vi "Simulated_Robot_Diff_Drive.vi"() -> ()   [LabVIEW 2019]
doc: "This WebSockets API example VI acts as a server for an incoming websockets connection. Receives/sends string data to the connected client."
uses:
  <vilib>/Rock Robotics/WPI/Simulation/Protocol/Devices/PWM/PWM proto.ctl
  <vilib>/Rock Robotics/WPI/Simulation/Protocol/Devices/PWM/PWM data proto.ctl
  <vilib>/Rock Robotics/WPI/Simulation/Protocol/Devices/RoboRIO/RoboRIO proto.ctl
  <vilib>/Rock Robotics/WPI/Simulation/Protocol/Devices/RoboRIO/RoboRIO data proto.ctl
  <vilib>/Rock Robotics/WPI/Simulation/Protocol/Devices/DriverStation/DS proto.ctl
  <vilib>/Rock Robotics/WPI/Simulation/Protocol/Devices/DriverStation/DS data proto.ctl
  <vilib>/Rock Robotics/WPI/Simulation/Protocol/Devices/Gyro/Gyro proto.ctl
  <vilib>/Rock Robotics/WPI/Simulation/Protocol/Devices/Gyro/Gyro Data proto.ctl
  <vilib>/Rock Robotics/WPI/Simulation/Protocol/Devices/Encoder/Encoder proto.ctl
  <vilib>/Rock Robotics/WPI/Simulation/Protocol/Devices/Encoder/Encoder data protoo.ctl
  <vilib>/Rock Robotics/WPI/ThirdParty/JAS_Junk/TrajLib/TypeDef/DIFF_DRIVE_TRAIN_SIM.ctl
  <vilib>/Rock Robotics/WPI/ThirdParty/JAS_Junk/TrajLib/TypeDef/LINEAR_SYSTEM.ctl
  <vilib>/Analysis/Matrix/Datatypes/RealMatrix.ctl
  <vilib>/Rock Robotics/WPI/ThirdParty/JAS_Junk/TrajLib/TypeDef/DCMOTOR.CTL
  <vilib>/vision/Image Controls.llb/IMAQ Image.ctl
  Simulated_Field/Simulated_Field_ROBOT_PICTURE.ctl
  DiffDriveSim/DiffDriveSim_PhysRobotInfoType.ctl
  DiffDriveSim/DiffDriveSim_KitBotDriveInfoType.ctl
  <vilib>/Rock Robotics/WPI/ThirdParty/JAS_Junk/TrajLib/Enum/DIFF_DRIVE_ToughBoxMini_MotorChoice_ENUM.ctl
  <vilib>/Rock Robotics/WPI/ThirdParty/JAS_Junk/TrajLib/Enum/DIFF_DRIVE_KitBot_WheelSize_ENUM.ctl
  <vilib>/Rock Robotics/WPI/ThirdParty/JAS_Junk/TrajLib/Enum/DIFF_DRIVE_ToughBoxMini_GearChoice_ENUM.ctl
  DiffDriveSim/DiffDriveSim_CustomDriveIntoType.ctl
  <vilib>/Rock Robotics/WPI/ThirdParty/JAS_Junk/TrajLib/Enum/DCMOTOR_TYPES_ENUM.ctl
  DiffDriveSim/DiffDriveSim_EncoderDIOType.ctl
  <vilib>/Rock Robotics/SystemInterfaces/DIO/FPGA_DIOChannel.ctl
  <vilib>/Rock Robotics/SystemInterfaces/DIO/FPGA_DIOPWMChannel.ctl
  <vilib>/Utility/miscctls.llb/LVBoundsTypeDef.ctl
  <vilib>/Rock Robotics/WPI/Simulation/Protocol/Devices/RoboRIO/RoboRIO Update Ops.ctl
  <vilib>/Rock Robotics/WPI/Simulation/Protocol/Devices/DriverStation/DS Update Ops.ctl
  <vilib>/Rock Robotics/WPI/ThirdParty/JAS_Junk/TrajLib/Rotation2d_CreateAngle.vi
  <vilib>/Rock Robotics/WPI/ThirdParty/JAS_Junk/TrajLib/Translation2d_Create.vi
  <vilib>/Rock Robotics/WPI/ThirdParty/JAS_Junk/TrajLib/MathUtil_Clamp.vi
  <vilib>/Rock Robotics/WPI/ThirdParty/JAS_Junk/TrajLib/BatterySim_CalculateLoadedBatteryVoltage.vi
  Simulated_Field/Simulated_Field_FIELD_ODOM_CLAMP.vi
  DiffDriveSim/DiffDriveSim_ClampFieldPosition.vi
  <vilib>/Rock Robotics/WPI/ThirdParty/JAS_Junk/TrajLib/Conv_Meters_Feet.vi
  DiffDriveSim/DiffDriveSim_FindEncoder.vi
  DiffDriveSim/DiffDriveSim_GetAllEncoderInx.vi
  <vilib>/Rock Robotics/SystemInterfaces/FPGA_NIFPGAInterfaceFPGAResourceConstant.vi
  <vilib>/MediaMongrels Ltd/WebSockets/WebSockets/WebSocket Server/WebSocket Server.lvclass
  C:/Program Files/National Instruments/LabVIEW 2019/vi.lib/MediaMongrels Ltd/WebSockets/WebSockets/WebSocket/WebSocket.lvclass
  Simulated_Robot_Globals.vi
  <vilib>/picture/pixmap.llb/Flatten Pixmap.vi
  <vilib>/picture/pictutil.llb/Create Mask.vi
  <vilib>/picture/picture.llb/Draw Flattened Pixmap.vi
  <vilib>/Rock Robotics/WPI/ThirdParty/JAS_Junk/TrajLib/DiffDriveTrainSim_SetInputs.vi
  <vilib>/Rock Robotics/WPI/ThirdParty/JAS_Junk/TrajLib/DiffDriveTrainSim_Update.vi
  <vilib>/Rock Robotics/WPI/ThirdParty/JAS_Junk/TrajLib/DiffDriveTrainSim_GetPose.vi
  <vilib>/Rock Robotics/WPI/ThirdParty/JAS_Junk/TrajLib/DiffDriveTrainSim_GetCurrentDrawAmps.vi
  <vilib>/Rock Robotics/WPI/ThirdParty/JAS_Junk/TrajLib/DiffDriveTrainSim_GetLeftVelocityMetersPerSecond.vi
  <vilib>/Rock Robotics/WPI/ThirdParty/JAS_Junk/TrajLib/DiffDriveTrainSim_GetRightPositionMeters.vi
  <vilib>/Rock Robotics/WPI/ThirdParty/JAS_Junk/TrajLib/DiffDriveTrainSim_GetLeftPositionMeters.vi
  <vilib>/Rock Robotics/WPI/ThirdParty/JAS_Junk/TrajLib/DiffDriveTrainSim_GetHeading.vi
  <vilib>/Rock Robotics/WPI/ThirdParty/JAS_Junk/TrajLib/DiffDriveTrainSim_GetRightVelocityMetersPerSecond.vi
  Simulated_Field/Simulated_Field.lvlib
  <vilib>/Rock Robotics/WPI/ThirdParty/JAS_Junk/TrajLib/Trajectory_Library.lvlib
  <vilib>/Rock Robotics/WPI/Simulation/Protocol/Devices/PWM/PWM Update Ops.ctl
  <vilib>/Rock Robotics/WPI/Simulation/Protocol/Devices/Gyro/Gyro Update Ops.ctl
  <vilib>/Rock Robotics/WPI/Simulation/Protocol/Devices/Encoder/Encoder Update Ops.ctl
  <vilib>/Analysis/Matrix/NI_Matrix.lvlib
panel:
  in  "Tab Control":T1(tab)
  out "Simulation\n  Running":bool
  in  "Start Simulation":bool
  in  "Field Selector":string(combo)
  in  "Robot Y Position\nInches":dbl=84.0
  in  "Robot X Position\nInches":dbl=120.0
  in  "Robot Orientation\nDegrees":dbl
  in  "Custom Drive Info":T2={"Motor Type"=enum."CIM", "Num Motors Per Side"=1, "Wheel Diameter Inch"=7.0, "Gear Ratio"=1.0} {"Gear Ratio" format="%#_13g"; "Wheel Diameter Inch" format="%#_13g"}
  in  "Robot Physical Info":T4={"Mass_LB"=80.0, "Actual TrackWidth Inch"=26.0, "Skid Factor"=1.75} {"Actual TrackWidth Inch" format="%#_13g"}
  in  "KitBot Drive Info":T5={"ToughBoxMiniMotor"=enum."One CIM Per Side", "Wheelsize"=enum."6 Inch", "ToughBoxMiniGear"=enum."Ratio_8_45"}
  in  "Use Custom Drive":bool
  in  "Encoder Counts/Rev":dbl=360.0
  in  "Left Drive Encoder":T9={"Enc A DI Channel"=enum."DIO 4", "Enc B DI Channel"=enum."DIO 5"}
  in  "Right Drive Encoder":T9={"Enc A DI Channel"=enum."DIO 6", "Enc B DI Channel"=enum."DIO 7"}
  in  "Left Drive Motor":T11
  in  "Right Drive Motor":T11=enum."PWM 1"
  out "Simulation\n  Running":bool
  out "Right Dist Ft":dbl format="%15.1f"
  out "Left Dist Ft":dbl format="%15.1f"
  out "Heading Deg":dbl format="%11.1f"
  out "Right Wheel\nFt / Sec":dbl format="%11.1f"
  out "Left Wheel\nFt / Sec":dbl format="%11.1f"
  out "RSL ON":picture
  out "ROBOT":T12
  out "RSL OFF":picture
  out "Field Picture":picture
  out "Y Pos Inch":dbl format="%11.1f"
  out "X Pos Inch":dbl format="%11.1f"
  out "Gyro":T13={"type"="Gyro", "device"="", "name"="", "data"={"<init"=0, ">connected"=FALSE, "<offsetX"=0.0, "<offsetY"=0.0, "<offsetZ"=0.0, ">angle_x"=0.0, ">angle_y"=0.0, ">angle_z"=0.0, ">rate_x"=0.0, ">rate_y"=0.0, ">rate_z"=0.0, "<gain"=0.0}}
  out "Enc Left":T15={"type"="Encoder", "device"="", "name"="", "data"={"<init"=FALSE, ">count"=0.0, ">period"=0.0, "<samples_to_avg"=0, "<offset"=0.0, "<channel_a"=0, "<channel_b"=0}}
  out "Enc Right":T15={"type"="Encoder", "device"="", "name"="", "data"={"<init"=FALSE, ">count"=0.0, ">period"=0.0, "<samples_to_avg"=0, "<offset"=0.0, "<channel_a"=0, "<channel_b"=0}}
  out "PWM 0":T17
  out "PWM 1":T17
  out "roboRIO":T19={"type"="roboRIO", "device"="", "name"="", "data"={">fpga_button"=FALSE, ">vin_voltage"=0.0, ">vin_current"=0.0, ">6v_voltage"=0.0, ">6v_current"=0.0, ">6v_active"=FALSE, ">6v_faults"=0.0, ">5v_voltage"=0.0, ">5v_current"=0.0, ">5v_active"=FALSE, ">5v_faults"=0.0, ">3v3_voltage"=0.0, ">3v3_current"=0.0, ">3v3_active"=FALSE, ">3v3_faults"=0.0}}
  out "Driverstation":T21={"type"="Driverstation", "device"="", "name"="", "data"={">enabled"=FALSE, ">autonomous"=FALSE, ">test"=FALSE, ">estop"=FALSE, ">fms"=FALSE, ">ds"=FALSE, "<match_time"=0.0, ">station"="", ">game_data"=""}}
  out "Request URI":string
  out "HTTP Headers":variant
  out "No Robot Comm":bool
  out "Battery Voltage VDC":dbl format="%18.2f"
  out "Gyro Reading   Deg":dbl format="%19.3f"
  out "Edges/Feet":dbl
  out "out DiffDriveTrainSim":T23 {"m_Motor"."Jr_KgM2" format="%13.5p"; "m_Motor"."L_H" format="%13.5p"; "m_Motor"."Kt_NMPerAmp" format="%13.5p"; "m_Motor"."KvINV_RadPerSecPerVolt" format="%13.5p"; "m_Motor"."R_Ohms" format="%13.5p"; "m_Motor"."FreeSpeed_RadPerSec" format="%13.5p"; "m_Motor"."FreeCurrent_Amps" format="%13.5p"; "m_Motor"."StallCurrent_Amps" format="%13.5p"; "m_Motor"."StallTorque_NM" format="%13.5p"; "m_Motor"."nominalVoltage_Volts" format="%13.5p"}
  out "Speed Left  Ft/Sec":dbl format="%13.2f"
  out "Speed Right  Ft/Sec":dbl format="%13.2f"
  out "Amps":dbl
  out "PWM 0 Rate":dbl format="%19.3f"
  out "PWM 1 Rate":dbl format="%19.3f"
  out "FIeld Image":T27
  out "Y Pos Pixel":dbl format="%11.1f"
  out "X Pos Pixel":dbl format="%11.1f"
  in  "Restart":bool
  out "Ctrl Loop Offset MS":dbl
  out "Robot Enabled":bool
  # "Robot Position"
  # "Robot Speed / Distance"
  # "<States, 1>"
  # "<Outputs, 1>"
  # "<Inputs, 1>"
  # "<Outputs, 1>"
  # "<States,States>"
  # "<States,Inputs>"
  # "<Outputs,States>"
  # "<Outputs,Inputs>"
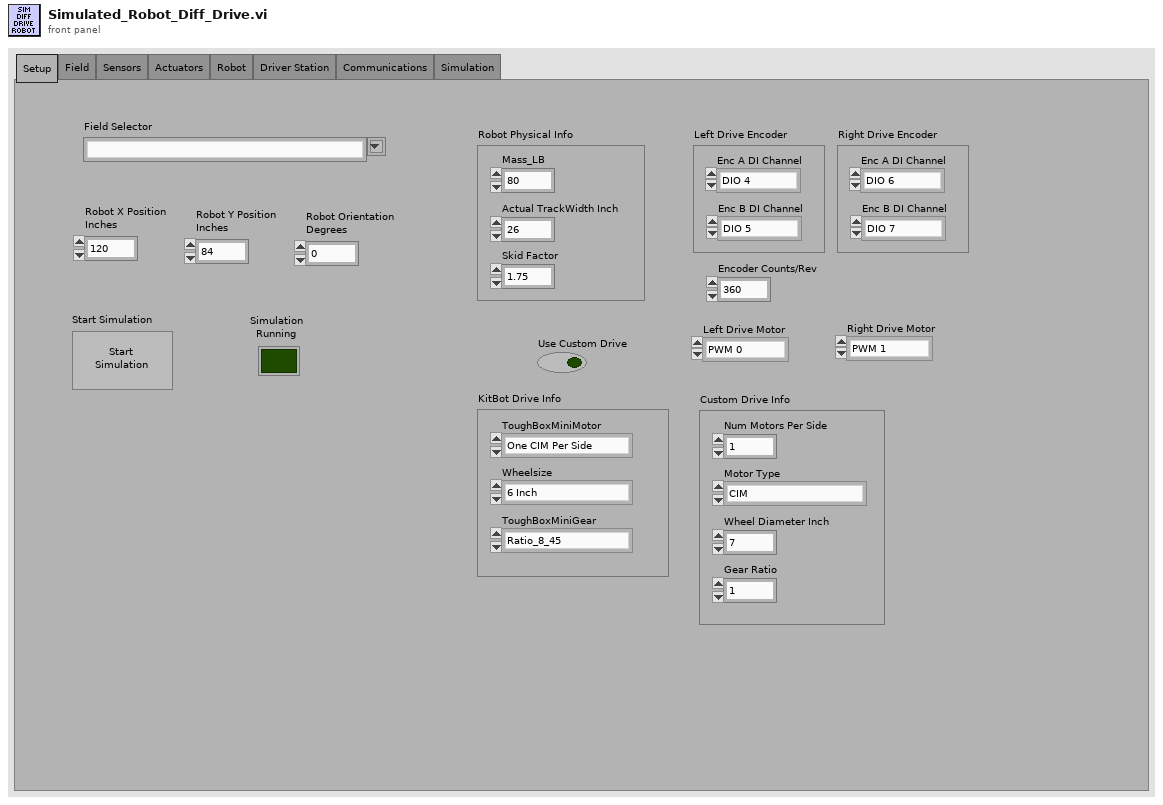
[diagram p1: front panel]
types:
  T1 = enum32{"Setup", "Field", "Sensors", "Actuators", "Robot", "Driver Station", "Communications", "Simulation"}
  T2 = typedef "DiffDriveSim_CustomDriveIntoType.ctl" = cluster{"Motor Type":T3, "Num Motors Per Side":i32, "Wheel Diameter Inch":dbl, "Gear Ratio":dbl}
  T3 = typedef "Trajectory_Library.lvlib/DCMOTOR_TYPES_ENUM.ctl" = enum16{"CIM", "AndyMark 9015", "Andy Mark RS 775 125", "Bag", "BaneBots RS 550", "BaneBots RS 775", "Falcon 500", "Mini CIM", "NEO", "NEO 550", "Romi BuiltIn", "Vex 775 Pro"}
  T4 = typedef "DiffDriveSim_PhysRobotInfoType.ctl" = cluster{"Mass_LB":dbl, "Actual TrackWidth Inch":dbl, "Skid Factor":dbl}
  T5 = typedef "DiffDriveSim_KitBotDriveInfoType.ctl" = cluster{"ToughBoxMiniMotor":T6, "Wheelsize":T7, "ToughBoxMiniGear":T8}
  T6 = typedef "Trajectory_Library.lvlib/DIFF_DRIVE_ToughBoxMini_MotorChoice_ENUM.ctl" = enum16{"One CIM Per Side", "Two CIM Per Side", "One MiniCIM Per Side", "Two Mini CIM Per Side", "Two Falcon Per Side", "Two NEO Per Side"}
  T7 = typedef "Trajectory_Library.lvlib/DIFF_DRIVE_KitBot_WheelSize_ENUM.ctl" = enum16{"4 Inch", "6 Inch", "8 Inch", "10 Inch"}
  T8 = typedef "Trajectory_Library.lvlib/DIFF_DRIVE_ToughBoxMini_GearChoice_ENUM.ctl" = enum16{"Ratio_12_75", "Ratio_10_71", "Ratio_8_45", "Ratio_7_31", "Ratio_5_95"}
  T9 = typedef "DiffDriveSim_EncoderDIOType.ctl" = cluster{"Enc A DI Channel":T10, "Enc B DI Channel":T10}
  T10 = typedef "FPGA_DIOChannel.ctl" = enum8{"DIO 0", "DIO 1", "DIO 2", "DIO 3", "DIO 4", "DIO 5", "DIO 6", "DIO 7", "DIO 8", "DIO 9", "DIO MXP 0", "DIO MXP 1", "DIO MXP 2", "DIO MXP 3", "DIO MXP 4", "DIO MXP 5", "DIO MXP 6", "DIO MXP 7", "DIO MXP 8", "DIO MXP 9", "DIO MXP 10", "DIO MXP 11", "DIO MXP 12", "DIO MXP 13", "DIO MXP 14", "DIO MXP 15", "SPI Port CS1", "SPI Port CS2", "SPI Port CS3", "SPI Port MISO", "SPI Port MOSI", "Invalid"}
  T11 = typedef "FPGA_DIOPWMChannel.ctl" = enum8{"PWM 0", "PWM 1", "PWM 2", "PWM 3", "PWM 4", "PWM 5", "PWM 6", "PWM 7", "PWM 8", "PWM 9", "PWM MXP 0", "PWM MXP 1", "PWM MXP 2", "PWM MXP 3", "PWM MXP 4", "PWM MXP 5", "PWM MXP 6", "PWM MXP 7", "PWM MXP 8", "PWM MXP 9", "Invalid"}
  T12 = typedef "Simulated_Field.lvlib/Simulated_Field_ROBOT_PICTURE.ctl" = picture
  T13 = typedef "Gyro proto.ctl" = cluster{"type":string, "device":string, "name":string, "data":T14}
  T14 = typedef "Gyro Data proto.ctl" = cluster{"<init":i32, ">connected":bool, "<offsetX":dbl, "<offsetY":dbl, "<offsetZ":dbl, ">angle_x":dbl, ">angle_y":dbl, ">angle_z":dbl, ">rate_x":dbl, ">rate_y":dbl, ">rate_z":dbl, "<gain":dbl}
  T15 = typedef "Encoder proto.ctl" = cluster{"type":string, "device":string, "name":string, "data":T16}
  T16 = typedef "Encoder data protoo.ctl" = cluster{"<init":bool, ">count":dbl, ">period":dbl, "<samples_to_avg":i32, "<offset":dbl, "<channel_a":i32, "<channel_b":i32}
  T17 = typedef "PWM proto.ctl" = cluster{"type":string, "device":string, "name":string, "data":T18}
  T18 = typedef "PWM data proto.ctl" = cluster{"<init":bool, "<speed":dbl, "<position":dbl, "<raw":dbl, "<period_scale":dbl, "<zero_latch":bool, "<servo range":dbl}
  T19 = typedef "RoboRIO proto.ctl" = cluster{"type":string, "device":string, "name":string, "data":T20}
  T20 = typedef "RoboRIO data proto.ctl" = cluster{">fpga_button":bool, ">vin_voltage":dbl, ">vin_current":dbl, ">6v_voltage":dbl, ">6v_current":dbl, ">6v_active":bool, ">6v_faults":dbl, ">5v_voltage":dbl, ">5v_current":dbl, ">5v_active":bool, ">5v_faults":dbl, ">3v3_voltage":dbl, ">3v3_current":dbl, ">3v3_active":bool, ">3v3_faults":dbl}
  T21 = typedef "DS proto.ctl" = cluster{"type":string, "device":string, "name":string, "data":T22}
  T22 = typedef "DS data proto.ctl" = cluster{">enabled":bool, ">autonomous":bool, ">test":bool, ">estop":bool, ">fms":bool, ">ds":bool, "<match_time":dbl, ">station":string, ">game_data":string}
  T23 = typedef "Trajectory_Library.lvlib/DIFF_DRIVE_TRAIN_SIM.ctl" = cluster{"m_Plant":T24, "m_X":T25, "m_Y":T25, "m_U":T25, "MeasureStdDev":T25, "m_Motor":T26, "m_OriginalGearing":dbl, "m_CurrentGearing":dbl, "m_WheelRadius_M":dbl, "m_RB":dbl}
  T24 = typedef "Trajectory_Library.lvlib/LINEAR_SYSTEM.ctl" = cluster{"m_A":T25, "m_B":T25, "m_C":T25, "m_D":T25, "States":i32, "Inputs":i32, "Outputs":i32}
  T25 = typedef "NI_Matrix.lvlib/RealMatrix.ctl" = dbl[][]
  T26 = typedef "Trajectory_Library.lvlib/DCMOTOR.CTL" = cluster{"nominalVoltage_Volts":dbl, "StallTorque_NM":dbl, "StallCurrent_Amps":dbl, "FreeCurrent_Amps":dbl, "FreeSpeed_RadPerSec":dbl, "R_Ohms":dbl, "KvINV_RadPerSecPerVolt":dbl, "Kt_NMPerAmp":dbl, "L_H":dbl, "Jr_KgM2":dbl}
  T27 = typedef "IMAQ Image.ctl" = refnum<image>
  T28 = typedef "LVBoundsTypeDef.ctl" = cluster{"Width":u32, "Height":u32}
  T29 = typedef "Image Type" = u32
  T30 = typedef "Simulated_Field.lvlib/Simulated_Field_Field_Info.ctl" = cluster{"FIeld_File_Name":string, "Top_Left_X":i32, "Top_Left_Y":i32, "Bottom_Right_X":i32, "Bottom_Right_Y":i32, "Field_Size_X":dbl, "Field_Size_Y":dbl, "FIeld_Size_Units":string}
  T31 = typedef "Trajectory_Library.lvlib/POSE2D.ctl" = cluster{"TRANSLATION":T32, "ROTATION":T33}
  T32 = typedef "Trajectory_Library.lvlib/TRANSLATION2D.ctl" = cluster{"X":dbl, "Y":dbl}
  T33 = typedef "Trajectory_Library.lvlib/ROTATION2D.ctl" = cluster{"VALUE":dbl, "COS":dbl, "SIN":dbl}
  T34 = typedef "DS Update Ops.ctl" = enum16{"set enabled", "set autonomous", "set test", "set estop", "set fms", "set ds", "set control word", "set match_time", "set station", "set game data", "JSON update", "set name", "get", "transmit initial", "reset"}
  T35 = typedef "RoboRIO Update Ops.ctl" = enum16{"get", "JSON update", "set name", "transmit initial", "set fpga_button", "set vin_voltage", "set vin_current", "set 6v_voltage", "set 6v_current", "set 6v_active", "set 6v_faults", "set 5v_voltage", "set 5v_current", "set 5v_active", "set 5v_faults", "set 3v3_voltage", "set 3v3_current", "set 3v3_active", "set 3v3_faults", "reset"}
  T36 = typedef "Simulated_Field.lvlib/Simulated_FIeld_Rotated_Picture_TypeDef.ctl" = cluster{"ONE-8-bit pixmap":u8[][], "Two-Array":cdb[][], "Three-Numeric":i32, "Four-Numeric":i32, "Five-Numeric":cdb, "Six-colors":u32[], "Seven-new element/subarray":u32, "Eight-Cluster":cluster{"[0]":i32, "[1]":i32}}
  T37 = typedef "DiffDriveSim_EncoderValues.ctl" = cluster{"Speed Ft/Sec":dbl, "Distance Ft":dbl}
  T38 = typedef "Encoder Update Ops.ctl" = enum16{"set init", "set count", "set period", "set reset", "set samples_to_avg", "get", "delete", "JSON update", "set name", "transmit initial", "reset", "set channel_a", "set channel_b", "set values"}
  T39 = typedef "Gyro Update Ops.ctl" = enum16{"get", "delete", "JSON update", "set  name", "transmit initial", "reset", "set init", "set offsetX", "set offsetY", "set offsetZ", "set gain", "set angle X", "set angle Y", "set angle Z", "set rate X", "set rate Y", "set rate Z"}
  T40 = typedef "PWM Update Ops.ctl" = enum16{"set init", "set speed", "set position", "set raw", "set  period_scale", "set zero_latch", "set angular range", "get", "delete", "JSON update", "set name", "transmit initial", "reset"}
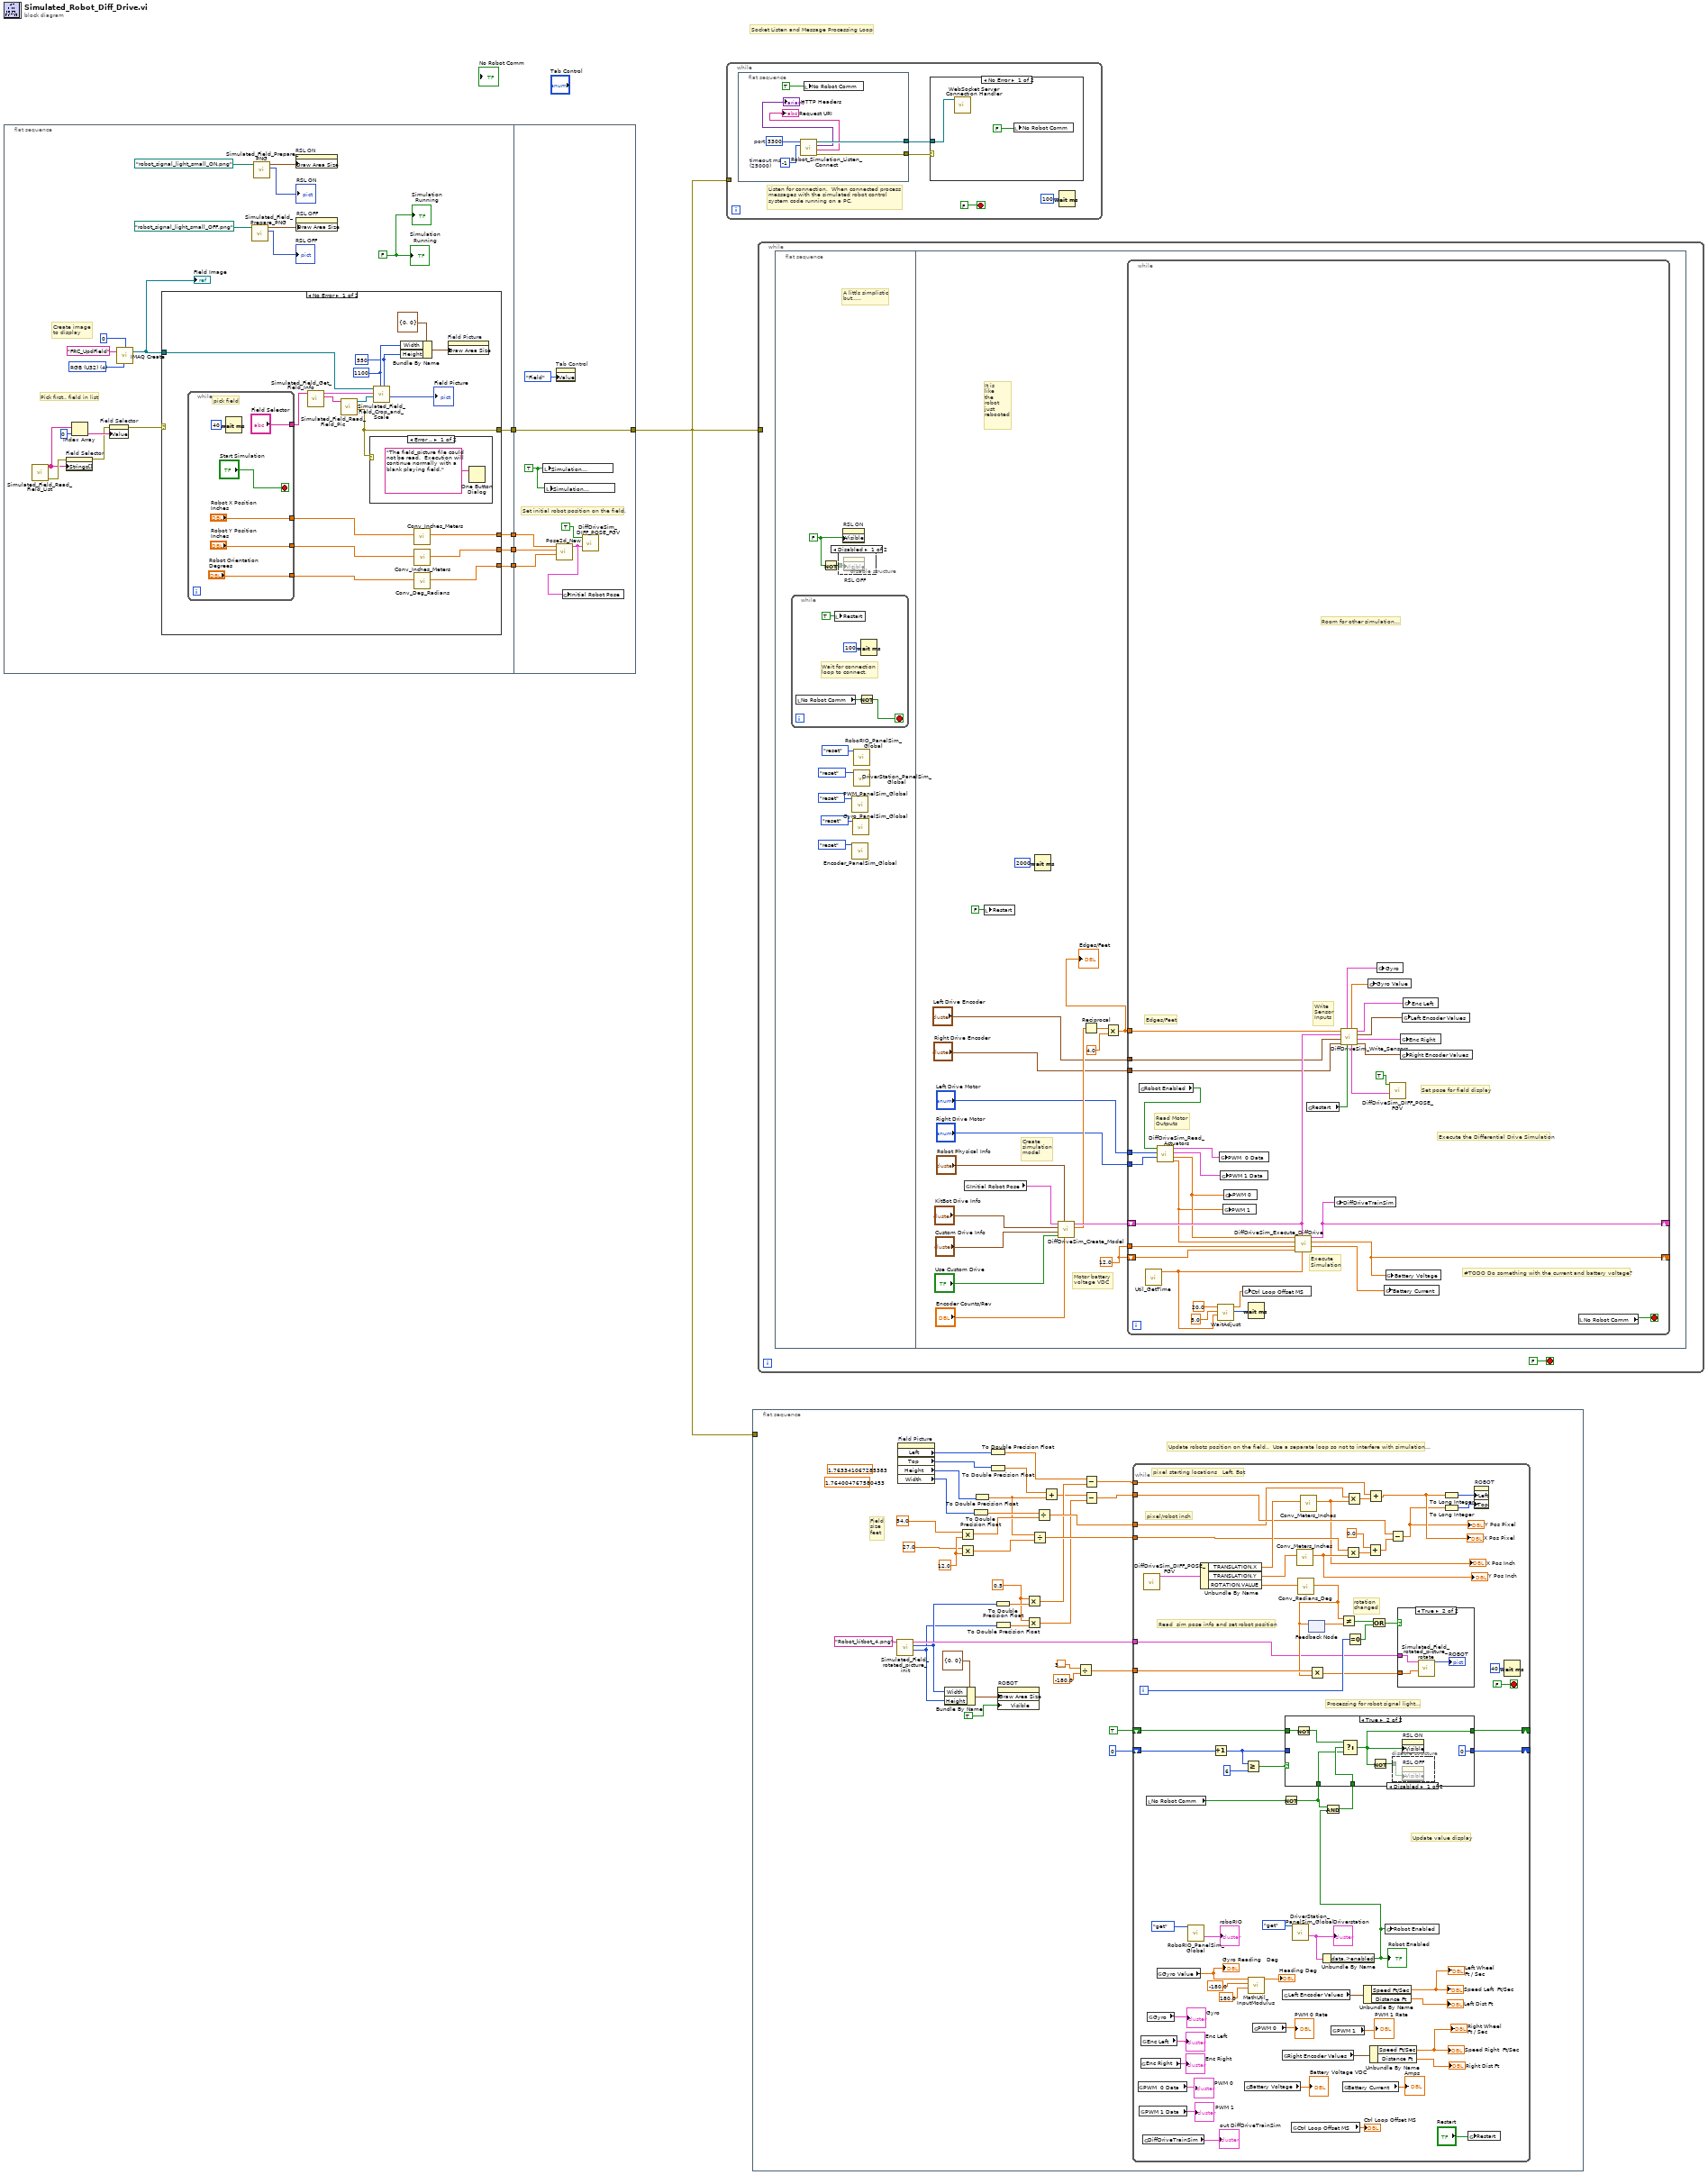
[diagram p0: block diagram]
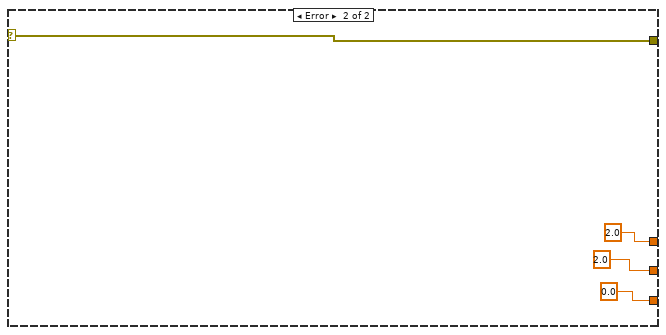
[diagram p6: hidden frame]
diagram:
  # "Socket Listen and Message Processing Loop"
  n1 = flat-sequence {
    tunnel: [w19] -> w5
    tunnel: [w9] -> w3
    tunnel: [w8] -> w2
    tunnel: [w7] -> w1
    tunnel: [w62] -> w4
    tunnel: w5 -> [w62]
    tunnel: w3 -> [w59]
    tunnel: w2 -> [w58]
    tunnel: w1 -> [w57]
    frame #0 {
      w6 = FALSE ("Simulation\n  Running")
      w24 = T29 4 items=["Grayscale (U8)", "Grayscale (I16)", "Grayscale (SGL)", "Complex (CSG)", "RGB (U32)", "HSL (U32)", "RGB (U64)", "Grayscale (U16)"] ("Image Type")
      # "Pick first.. field in list"
      # "Create image \nto display"
      n2 = call "Simulated_Field_Read_Field_List.vi"() -> ("error out"=w15:errorcluster, "section names"=w14:string[])  [unwired: 10 in]
      n3 = property on="Field Selector" class="CmbBox"(error in=w15, "Strings[]"=w14) -> (error out=w11:errorcluster)  [unwired: 1 in, 1 out]
      n4 = Index Array(array=w14, index=0) -> (element=w12:string)
      n5 = property on="Field Selector" class="CmbBox"(error in=w11, "Value"=w12) -> (error out=w10:errorcluster)  [unwired: 1 in, 1 out]
      n6 = call "IMAQ Create"("Border Size"=0, "Image Name"="FRC_UpdField", "Image Type"=w24) -> ("New Image"=w23:T27)  [unwired: 2 in, 1 out]
      "FIeld Image" <- w23
      n7 = case shown="No Error" w10 {
        selector: w10 -> [_ w54]
        tunnel: w23 -> [w34 _]
        tunnel: [w40 w54] -> w19
        tunnel: [w29 2.0 ("Meters")] -> w9
        tunnel: [w28 2.0 ("Meters")] -> w8
        tunnel: [w27 0.0 ("Radians")] -> w7
        frame No Error {
          w35 = 550 ("Disp Y Size Pixel")
          w36 = 1100 ("Disp X Size Pixel")
          n8 = while {
            tunnel: ["Field Selector"] -> w33
            tunnel: ["Robot X Position\nInches"] -> w32
            tunnel: ["Robot Y Position\nInches"] -> w31
            tunnel: ["Robot Orientation\nDegrees"] -> w30
            stop <- "Start Simulation" stop-if-true
            # "pick field"
            n9 = Wait (ms)(milliseconds to wait=u32 40) -> ()  [unwired: 1 out]
          }
          n10 = call "Simulated_Field_Get_Field_Info.vi"("Field Selector"=w33) -> ("File"=w43:string, "input cluster"=w42:T30)  [unwired: 9 in]
          n11 = call "Simulated_Field_Read_Field_Pic.vi"("file name"=w43) -> ("Image Error"=w40:errorcluster, "Image Data"=w41:T27)  [unwired: 7 in, 2 out]
          n12 = case shown="Error .." w40 {
            frame Error {
              n13 = One Button Dialog(message="The field_picture file could not be read.  Execution will continue normally with a blank playing field.") -> ()  [unwired: 1 in, 1 out]
            }
            frame No Error {
            }
          }
          n14 = call "Simulated_Field_Field_Crop_and_Scale.vi"("Disp Y Size Pixel"=w35, "Disp X Size Pixel"=w36, "Field Image"=w41, "field Info"=w42, "Display Image"=w34) -> ("Cropped Field Picture Out"=→"Field Picture":picture)  [unwired: 4 in, 2 out]
          n15 = Bundle By Name(cluster=T28 {"Width"=0, "Height"=0} ("Draw Area Size"), "Width"=w36, "Height"=w35) -> (w37:T28)
          n16 = call <vilib>:"Conv_Inches_Meters.vi"("INCH"=w32) -> ("Meters"=w29:dbl)  [unwired: 10 in]
          n17 = call <vilib>:"Conv_Inches_Meters.vi"("INCH"=w31) -> ("Meters"=w28:dbl)  [unwired: 10 in]
          n18 = call <vilib>:"Conv_Deg_Radians.vi"("Degress"=w30) -> ("Radians"=w27:dbl)  [unwired: 10 in]
          n19 = property on="Field Picture" class="Pict"("Draw Area Size"=w37) -> ()  [unwired: 2 in, 2 out]
        }
        frame Error {
        }
      }
      n20 = call "Simulated_Field_Prepare_PNG.vi"("path to PNG file"=path "robot_signal_light_small_OFF.png") -> ("new picture"=→"RSL OFF":picture, "Draw Area Size"=w18:T28)  [unwired: 9 in]
      n21 = call "Simulated_Field_Prepare_PNG.vi"("path to PNG file"=path "robot_signal_light_small_ON.png") -> ("new picture"=→"RSL ON":picture, "Draw Area Size"=w21:T28)  [unwired: 9 in]
      n22 = property on="RSL ON" class="Pict"("Draw Area Size"=w21) -> ()  [unwired: 2 in, 2 out]
      n23 = property on="RSL OFF" class="Pict"("Draw Area Size"=w18) -> ()  [unwired: 2 in, 2 out]
      "Simulation\n  Running" <- w6
      "Simulation\n  Running" <- w6
    }
    frame #1 {
      w55 = TRUE ("Simulation\n  Running")
      # "Set initial robot position on the field."
      n24 = local write "Simulation\n  Running"(w55) -> ()
      n25 = local write "Simulation\n  Running"(w55) -> ()
      n26 = property on="Tab Control" class="TabCtl (strict)"("Value"=T1."Field" ("Tab Control")) -> ()  [unwired: 2 in, 2 out]
      n27 = call <vilib>:"Pose2d_New.vi"("Heading"=w57, "Y"=w58, "X"=w59) -> ("out POSe"=w56:T31)  [unwired: 8 in]
      n28 = global write "Simulated_Robot_Globals.vi" "Initial Robot Pose"(w56) -> ()
      n29 = call "DiffDriveSim_DIFF_POSE_FGV.vi"("in Sim Pose"=w56, "WRITE"=TRUE) -> ()  [unwired: 9 in, 1 out]
    }
  }
  n30 = while {
    tunnel: w4 -> [_]
    stop <- FALSE stop-if-true
    # "Listen for connection.  When connected process\nmessages with the simulated robot control\nsystem code running on a PC."
    n31 = flat-sequence {
      tunnel: [w71] -> w65
      tunnel: [w69] -> w64
      frame #0 {
        w72 = -1  # timeout ms  (25000)
        w73 = u16 3300  # port
        n32 = call <vilib>:"Robot_Simulation_Listen_Connect.vi"("timeout ms (25000)"=w72, "port"=w73) -> ("error out"=w71:errorcluster, "Properties:Request URI"=→"Request URI":string, "Properties:Return Headers"=→"HTTP Headers":variant, "WebSocket Connection out"=w69:refnum<class "WebSocket Server.lvclass">)  [unwired: 6 in]
        n33 = local write "No Robot Comm"(TRUE ("Stop\nSim")) -> ()
      }
    }
    n34 = case shown="No Error" w65 {
      tunnel: w64 -> [w74 _]
      frame No Error {
        n35 = call <vilib>:"WebSocket Server Connection Handler.vi"("WebSocket in"=w74) -> ()  [unwired: 10 in, 1 out]
        n36 = local write "No Robot Comm"(FALSE ("Stop\nSim")) -> ()
      }
      frame Error {
      }
    }
    n37 = Wait (ms)(milliseconds to wait=u32 100) -> ()  [unwired: 1 out]
  }
  n38 = flat-sequence {
    tunnel: w4 -> [_]
    frame #0 {
      w88 = 0.5
      (unwired) 1.764004767580453
      (unwired) 1.763341067285383
      w106 = 12.0 ("y")
      # "Field\nsize\nfeet"
      # "Update robots position on the field..  Use a separate loop so not to interfere with simulation..."
      n39 = call "Simulated_Field_rotated_picture_init.vi"("Picture FIle Name"="Robot_kitbot_4.png") -> ("Height"=w80:i16, "Width"=w81:i16, "RotatedPictureInfo"=w107:T36)  [unwired: 7 in, 1 out]
      n40 = property on="Field Picture" class="Pict"() -> ("Left"=w103:i32, "Top"=w102:i32, "Height"=w101:u32, "Width"=w100:u32)  [unwired: 2 in, 2 out]
      n41 = Bundle By Name(cluster=T28 {"Width"=0, "Height"=0} ("Draw Area Size"), "Width"=w81, "Height"=w80) -> (w83:T28)
      n42 = Multiply(x=54.0, y=w106) -> (x*y=w97:dbl)
      n43 = Multiply(x=27.0, y=w106) -> (x*y=w94:dbl)
      n44 = To Double Precision Float(number=w100) -> (double precision float=w98:dbl)
      n45 = To Double Precision Float(number=w101) -> (double precision float=w95:dbl)
      n46 = To Double Precision Float(number=w103) -> (double precision float=w87:dbl)
      n47 = To Double Precision Float(number=w102) -> (double precision float=w99:dbl)
      n48 = To Double Precision Float(number=w81) -> (double precision float=w90:dbl)
      n49 = To Double Precision Float(number=w80) -> (double precision float=w89:dbl)
      n50 = property on="ROBOT" class="Pict (strict)"("Draw Area Size"=w83, "Visible"=TRUE) -> ()  [unwired: 2 in, 2 out]
      n51 = Multiply(x=w88, y=w90) -> (x*y=w86:dbl)
      n52 = Multiply(x=w88, y=w89) -> (x*y=w84:dbl)
      n53 = Divide(x=w95, y=w94) -> (x/y=w93:dbl)
      n54 = Divide(x=w98, y=w97) -> (x/y=w96:dbl)
      n55 = Add(x=w99, y=w95) -> (x+y=w85:dbl)
      n56 = Divide(x=3.141592653589793, y=-180.0 ("value")) -> (x/y=w110:dbl)
      n57 = Subtract(x=w87, y=w86) -> (x-y=w92:dbl)
      n58 = Subtract(x=w85, y=w84) -> (x-y=w91:dbl)
      n59 = while {
        tunnel: w110 -> [w176]
        tunnel: w107 -> [w159]
        tunnel: w92 -> [w158]
        tunnel: w91 -> [w157]
        tunnel: w96 -> [w156]
        tunnel: w93 -> [w155]
        shift-right: [w141] -> _
        shift-left: 0 -> [w144]
        shift-right: [w142] -> _
        shift-left: TRUE -> [w143]
        i -> [w165]
        stop <- FALSE stop-if-true
        # "Update value display"
        # "Processing for robot signal light..."
        # "pixel starting locations   Left, Bot"
        # "Read  sim pose info and set robot position"
        # "pixel/robot inch"
        # "rotation\nchanged"
        n60 = global read "Simulated_Robot_Globals.vi" "PWM  0 Data"() -> (→"PWM 0":T17)
        n61 = global read "Simulated_Robot_Globals.vi" "PWM 1 Data"() -> (→"PWM 1":T17)
        n62 = global read "Simulated_Robot_Globals.vi" "Enc Right"() -> (→"Enc Right":T15)
        n63 = global read "Simulated_Robot_Globals.vi" "Enc Left"() -> (→"Enc Left":T15)
        n64 = global read "Simulated_Robot_Globals.vi" "DiffDriveTrainSim"() -> (→"out DiffDriveTrainSim":T23)
        n65 = call "DiffDriveSim_DIFF_POSE_FGV.vi"() -> ("out Sim Pose"=w148:T31)  [unwired: 11 in]
        n66 = local read "No Robot Comm"() -> (w111:bool)
        n67 = global read "Simulated_Robot_Globals.vi" "Gyro"() -> (→"Gyro":T13)
        n68 = global read "Simulated_Robot_Globals.vi" "Gyro Value"() -> (w131:dbl)
        "Gyro Reading   Deg" <- w131
        n69 = call <vilib>:"RoboRIO_PanelSim_Global.vi"("Menu"=RoboRIO_Update_Ops."get") -> ("roboRIO new"=→"roboRIO":T19)  [unwired: 13 in, 1 out]
        n70 = Unbundle By Name(w148) -> ("TRANSLATION.X"=w164:dbl, "TRANSLATION.Y"=w163:dbl, "ROTATION.VALUE"=w161:dbl)
        n71 = Increment(x=w144) -> (x+1=w146:i32)
        n72 = global read "Simulated_Robot_Globals.vi" "Battery Voltage"() -> (→"Battery Voltage VDC":dbl)
        n73 = Greater Or Equal?(x=w146, y=6) -> (x >= y?=w147:bool)
        n74 = call <vilib>:"MathUtil_InputModulus.vi"("Maximum_Input"=180.0, "Minimum_Input"=-180.0, "Input"=w131) -> ("modulus"=→"Heading Deg":dbl)  [unwired: 8 in]
        n75 = global read "Simulated_Robot_Globals.vi" "PWM 0"() -> (→"PWM 0 Rate":dbl)
        n76 = global read "Simulated_Robot_Globals.vi" "Right Encoder Values"() -> (w119:T37)
        n77 = global read "Simulated_Robot_Globals.vi" "Left Encoder Values"() -> (w120:T37)
        n78 = Not(x=w111) -> (.not. x?=w139:bool)
        n79 = global read "Simulated_Robot_Globals.vi" "Ctrl Loop Offset MS"() -> (→"Ctrl Loop Offset MS":dbl)
        n80 = call <vilib>:"DriverStation_PanelSim_Global.vi"("menu"=DS_Update_Ops."get") -> ("Driverstation new"=w136:T21)  [unwired: 13 in, 1 out]
        "Driverstation" <- w136
        n81 = call <vilib>:"Conv_Meters_Inches.vi"("Meters"=w163) -> ("Inches"=w150:dbl)  [unwired: 10 in]
        "Y Pos Inch" <- w150
        n82 = call <vilib>:"Conv_Radians_Deg.vi"("Radians"=w161) -> ("Degrees"=w162:dbl)  [unwired: 10 in]
        n83 = call <vilib>:"Conv_Meters_Inches.vi"("Meters"=w164) -> ("Inches"=w149:dbl)  [unwired: 10 in]
        "X Pos Inch" <- w149
        n84 = feedback-in #1(w162) -> ()
        n85 = feedback #1() -> (w173:dbl)  [unwired: 1 in]
        n86 = Multiply(x=w176, y=w162) -> (x*y=w160:dbl)
        n87 = Unbundle By Name(w136) -> ("data.>enabled"=w112:bool)
        "Robot Enabled" <- w112
        n88 = And(x=w139, y=w112) -> (x .and. y?=w140:bool)
        n89 = case shown="True" w147 {
          tunnel: w143 -> [w178 w185]
          tunnel: [w178 w181] -> w142
          tunnel: w146 -> [w177 _]
          tunnel: [w177 0] -> w141
          tunnel: w140 -> [_ w183]
          tunnel: w139 -> [_ w179]
          frame False {
          }
          frame True {
            n90 = Not(x=w185) -> (.not. x?=w184:bool)
            n91 = Select(t=w184, s=w183, f=w179) -> (s? t:f=w181:bool)
            n92 = Not(x=w181) -> (.not. x?=w182:bool)
            n93 = disable-structure shown="Disabled" {
              disable-tunnel: w182 -> [w186 _]
              frame Disabled {
                n94 = property on="RSL OFF" class="Pict"("Visible"=w186) -> ()  [unwired: 2 in, 2 out]
              }
              frame Enabled {
              }
            }
            n95 = property on="RSL ON" class="Pict"("Visible"=w181) -> ()  [unwired: 2 in, 2 out]
          }
        }
        n96 = global read "Simulated_Robot_Globals.vi" "PWM 1"() -> (→"PWM 1 Rate":dbl)
        n97 = Not Equal?(x=w162, y=w173) -> (x != y?=w167:bool)
        n98 = global read "Simulated_Robot_Globals.vi" "Battery Current"() -> (→"Amps":dbl)
        n99 = Multiply(x=w155, y=w150) -> (x*y=w171:dbl)
        n100 = Multiply(x=w156, y=w149) -> (x*y=w172:dbl)
        n101 = Equal To 0?(x=w165) -> (x = 0?=w166:bool)
        n102 = Unbundle By Name(w120) -> ("Speed Ft/Sec"=→"Speed Left  Ft/Sec" →"Left Wheel\nFt / Sec":dbl, "Distance Ft"=→"Left Dist Ft":dbl)
        n103 = Add(x=0.0, y=w171) -> (x+y=w169:dbl)
        n104 = Add(x=w158, y=w172) -> (x+y=w152:dbl)
        "X Pos Pixel" <- w152
        n105 = Unbundle By Name(w119) -> ("Speed Ft/Sec"=→"Speed Right  Ft/Sec" →"Right Wheel\nFt / Sec":dbl, "Distance Ft"=→"Right Dist Ft":dbl)
        n106 = Or(x=w167, y=w166) -> (x .or. y?=w168:bool)
        n107 = global write "Simulated_Robot_Globals.vi" "Robot Enabled"(w112) -> ()
        n108 = Subtract(x=w157, y=w169) -> (x-y=w151:dbl)
        "Y Pos Pixel" <- w151
        n109 = case shown="True" w168 {
          tunnel: w160 -> [_ w187]
          tunnel: w159 -> [_ w188]
          frame False {
          }
          frame True {
            n110 = call "Simulated_Field_rotated_picture_rotate.vi"("Angle"=w187, "RotatedPictureInfo"=w188) -> ("new picture"=→"ROBOT":picture)  [unwired: 9 in]
          }
        }
        n111 = To Long Integer(number=w152) -> (32bit integer=w154:i32)
        n112 = To Long Integer(number=w151) -> (32bit integer=w153:i32)
        n113 = global write "Simulated_Robot_Globals.vi" "Restart"("Restart") -> ()
        n114 = property on="ROBOT" class="Pict (strict)"("Left"=w154, "Top"=w153) -> ()  [unwired: 2 in, 2 out]
        n115 = Wait (ms)(milliseconds to wait=u32 40) -> ()  [unwired: 1 out]
      }
    }
  }
  n116 = while {
    tunnel: w4 -> [_]
    stop <- FALSE stop-if-true
    n117 = flat-sequence {
      frame #0 {
        w196 = FALSE ("Visible")
        # "A littls simplistic\nbut....."
        n118 = while {
          stop <- w200 stop-if-true
          # "Wait for connection\nloop to connect."
          n119 = local read "No Robot Comm"() -> (w201:bool)
          n120 = local write "Restart"(TRUE ("Restart")) -> ()
          n121 = Not(x=w201) -> (.not. x?=w200:bool)
          n122 = Wait (ms)(milliseconds to wait=u32 100) -> ()  [unwired: 1 out]
        }
        n123 = Not(x=w196) -> (.not. x?=w197:bool)
        n124 = disable-structure shown="Disabled" {
          disable-tunnel: w197 -> [w198 _]
          frame Disabled {
            n125 = property on="RSL OFF" class="Pict"("Visible"=w198) -> ()  [unwired: 2 in, 2 out]
          }
          frame Enabled {
          }
        }
        n126 = property on="RSL ON" class="Pict"("Visible"=w196) -> ()  [unwired: 2 in, 2 out]
        n127 = call <vilib>:"PWM_PanelSim_Global.vi"("menu"=PWM_Update_Ops."reset") -> ()  [unwired: 13 in, 2 out]
        n128 = call <vilib>:"Encoder_PanelSim_Global.vi"("menu"=Encoder_Update_Ops."reset") -> ()  [unwired: 13 in, 2 out]
        n129 = call <vilib>:"Gyro_PanelSim_Global.vi"("Menu"=Gyro_Update_Ops."reset") -> ()  [unwired: 13 in, 2 out]
        n130 = call <vilib>:"RoboRIO_PanelSim_Global.vi"("Menu"=RoboRIO_Update_Ops."reset") -> ()  [unwired: 13 in, 2 out]
        n131 = call <vilib>:"DriverStation_PanelSim_Global.vi"("menu"=DS_Update_Ops."reset") -> ()  [unwired: 13 in, 2 out]
      }
      frame #1 {
        w219 = 12.0 ("Voltage")
        # "Create\nsimulation\nmodel"
        # "Motor battery\nvoltage VDC"
        # "It is\nlike\nthe \nrobot \njust\nrebooted"
        n132 = global read "Simulated_Robot_Globals.vi" "Initial Robot Pose"() -> (w203:T31)
        n133 = local write "Restart"(FALSE ("Restart")) -> ()
        n134 = Wait (ms)(milliseconds to wait=u32 2000) -> ()  [unwired: 1 out]
        n135 = call "DiffDriveSim_Create_Model.vi"("Encoder Counts/Rev"="Encoder Counts/Rev", "Robot Physical Info"="Robot Physical Info", "Use Custom Drive"="Use Custom Drive", "Custom Drive Info"="Custom Drive Info", "KitBot Drive Info"="KitBot Drive Info", "Initial Robot Position"=w203) -> ("Encoder Ft/Count"=w218:dbl, "out DiffDriveTrainSim"=w220:T23)  [unwired: 4 in]
        n136 = Reciprocal(x=w218) -> (1/x=w212:dbl)
        n137 = Multiply(x=w212, y=4.0) -> (x*y=w210:dbl)
        "Edges/Feet" <- w210
        n138 = while {
          shift-right: [w225] -> _
          shift-left: w220 -> [w248]
          shift-right: [w232] -> _
          shift-left: w219 -> [w246]
          tunnel: w210 -> [w249]
          tunnel: w219 -> [w247]
          tunnel: "Left Drive Encoder" -> [w244]
          tunnel: "Right Drive Encoder" -> [w243]
          tunnel: "Left Drive Motor" -> [w242]
          tunnel: "Right Drive Motor" -> [w241]
          stop <- w251 stop-if-true
          # "Room for other simulation..."
          # "Execute\nSimulation"
          # "Write\nSensor\nInputs"
          # "Read Motor\nOutputs"
          # "#TODO Do something with the current and battery voltage?"
          # "Edges/Feet"
          # "Set pose for field display"
          # "Execute the Differential Drive Simulation"
          n139 = global read "Simulated_Robot_Globals.vi" "Robot Enabled"() -> (w236:bool)
          n140 = call <vilib>:"Util_GetTime.vi"() -> ("FPGA_Time_Seconds"=w237:dbl)  [unwired: 10 in, 1 out]
          n141 = call "DiffDriveSim_Read_Actuators.vi"("Right Drive Motor"=w241, "Left Drive Motor"=w242, "Robot Enabled"=w236) -> ("Right Motor Dmd"=w233:dbl, "Left Motor Dmd"=w234:dbl, "Right PWM Sim"=w221:T17, "Left PWM Sim"=w222:T17)  [unwired: 5 in]
          n142 = call <vilib>:"WaitAdjust.vi"("Time_SEC"=w237, "MaxDeviation_MS"=5.0, "DesiredLoopTime_MS"=20.0) -> ("AdjustedWaitTime_MS"=w238:u32, "Offset_MS"=w230:dbl)  [unwired: 7 in]
          n143 = global write "Simulated_Robot_Globals.vi" "PWM  0 Data"(w222) -> ()
          n144 = global write "Simulated_Robot_Globals.vi" "PWM 1 Data"(w221) -> ()
          n145 = global write "Simulated_Robot_Globals.vi" "PWM 1"(w233) -> ()
          n146 = global write "Simulated_Robot_Globals.vi" "PWM 0"(w234) -> ()
          n147 = global write "Simulated_Robot_Globals.vi" "Ctrl Loop Offset MS"(w230) -> ()
          n148 = Wait (ms)(milliseconds to wait=w238) -> ()  [unwired: 1 out]
          n149 = call "DiffDriveSim_Execute_DiffDrive.vi"("Time"=w237, "in DiffDriveTrainSim"=w248, "Actual  Battery Voltage"=w246, "Nominal Battery Voltage"=w247, "Right Motor Dmd"=w233, "Left Motor Dmd"=w234) -> ("Current Amps"=w231:dbl, "Battery Volts"=w232:dbl, "out DiffDriveTrainSim"=w225:T23)  [unwired: 3 in]
          n150 = global read "Simulated_Robot_Globals.vi" "Restart"() -> (w235:bool)
          n151 = global write "Simulated_Robot_Globals.vi" "DiffDriveTrainSim"(w225) -> ()
          n152 = call "DiffDriveSim_Write_Sensors.vi"("Restart"=w235, "Right Encoder"=w243, "Left Encoder"=w244, "Diff Drive Train Sim"=w248, "Counts/Feet"=w249) -> (0:"Right Encoder"=w228:T37, 1:"Right Encoder"=w226:T15, 2:"Left Encoder"=w229:T37, 3:"Left Encoder"=w227:T15, "Robot Pose"=w245:T31, "Gyro Deg"=w223:dbl, "Gyro"=w224:T13)
          n153 = global write "Simulated_Robot_Globals.vi" "Gyro Value"(w223) -> ()
          n154 = global write "Simulated_Robot_Globals.vi" "Gyro"(w224) -> ()
          n155 = global write "Simulated_Robot_Globals.vi" "Battery Current"(w231) -> ()
          n156 = global write "Simulated_Robot_Globals.vi" "Battery Voltage"(w232) -> ()
          n157 = call "DiffDriveSim_DIFF_POSE_FGV.vi"("in Sim Pose"=w245, "WRITE"=TRUE) -> ()  [unwired: 9 in, 1 out]
          n158 = global write "Simulated_Robot_Globals.vi" "Enc Right"(w226) -> ()
          n159 = global write "Simulated_Robot_Globals.vi" "Right Encoder Values"(w228) -> ()
          n160 = global write "Simulated_Robot_Globals.vi" "Left Encoder Values"(w229) -> ()
          n161 = global write "Simulated_Robot_Globals.vi" "Enc Left"(w227) -> ()
          n162 = local read "No Robot Comm"() -> (w251:bool)
        }
      }
    }
  }
